vi "test_Move to 0 with Return Speed.vi"(8 "error in (no error)":errorcluster, 11 "TestCase in":refnum<class "EM1000 Turn Table.lvclass">) -> (0 "error out":errorcluster, 3 "TestCase out":refnum<class "EM1000 Turn Table.lvclass">)   [LabVIEW 2020, in "EM1000 Turn Table.lvclass"]
uses:
  EM1000 Turn Table.lvclass
  EM1000 Turn Table.lvclass/EM1000 Turn Table.ctl
  <vilib>/addons/_JKI Toolkits/VI Tester/TestCase.llb/TestCase.lvclass
  AUDIX EM1000.lvclass
  C:/Program Files (x86)/National Instruments/LabVIEW 2020/vi.lib/addons/_JKI Toolkits/VI Tester/TestCase.llb/TestCase.lvclass
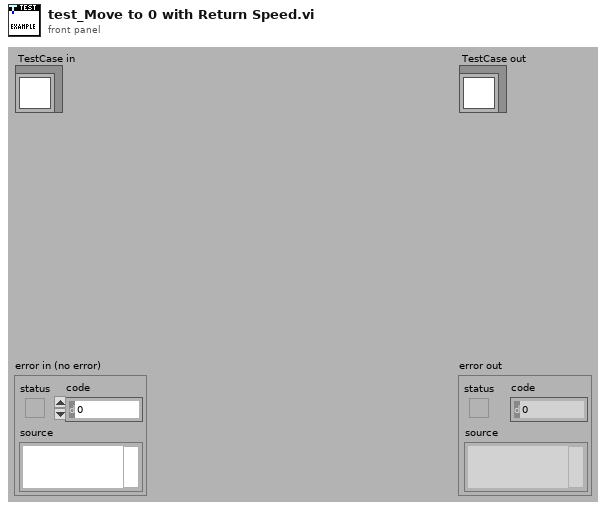
[diagram p1: front panel]
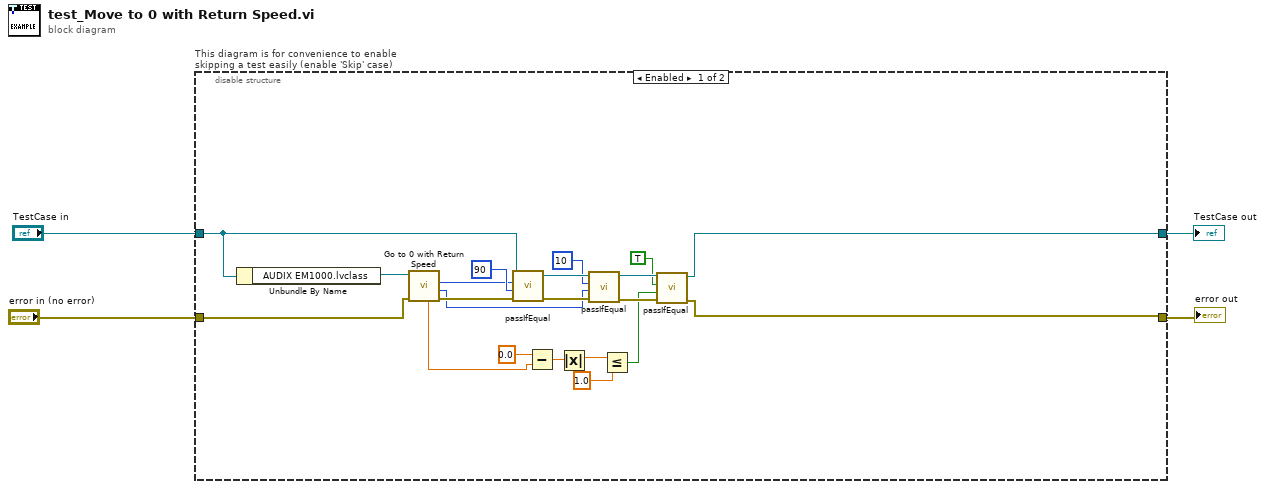
[diagram p0: block diagram]
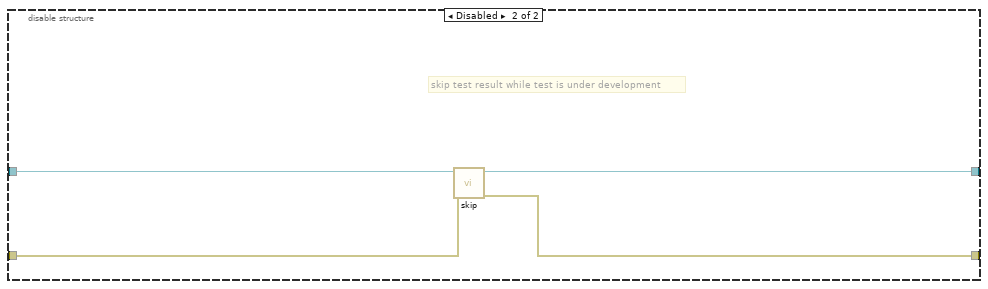
[diagram p2: hidden frame]
diagram:
  n1 = disable-structure "This diagram is for convenience to enable skipping a test easily (enable 'Skip' case)" shown="Enabled" {
    disable-tunnel: "TestCase in" -> [w19 w29]
    disable-tunnel: [w18 w27] -> w1
    disable-tunnel: [w17 w28] -> w3
    disable-tunnel: "error in (no error)" -> [w15 w26]
    frame Enabled {
      n2 = Unbundle By Name(w19) -> ("AUDIX EM1000.lvclass"=w16:refnum<class "AUDIX EM1000.lvclass">)
      n3 = call "Go to 0 with Return Speed.vi"("error in (no error)"=w15, "AUDIX EM1000 in"=w16) -> ("error out"=w14:errorcluster, "Final Speed"=w13:i32, "Return Speed"=w12:i32, "TT Angle"=w7:dbl)  [unwired: 5 in, 1 out]
      n4 = call-dynamic "passIfEqual.vi"("error in (no error)"=w14, "y"=90, "x"=w12, "TestCase in"=w19) -> ("error out"=w21:errorcluster, "TestCase out"=w24:refnum<class "EM1000 Turn Table.lvclass">)  [unwired: 6 in]
      n5 = Subtract(x=0.0, y=w7) -> (x-y=w9:dbl)
      n6 = Absolute Value(x=w9) -> (abs(x)=w10:dbl)
      n7 = call-dynamic "passIfEqual.vi"("error in (no error)"=w21, "y"=w13, "x"=10, "TestCase in"=w24) -> ("error out"=w20:errorcluster, "TestCase out"=w22:refnum<class "EM1000 Turn Table.lvclass">)  [unwired: 6 in]
      n8 = Less Or Equal?(x=w10, y=1.0) -> (x <= y?=w6:bool)
      n9 = call-dynamic "passIfEqual.vi"("error in (no error)"=w20, "y"=w6, "x"=TRUE, "TestCase in"=w22) -> ("error out"=w17:errorcluster, "TestCase out"=w18:refnum<class "EM1000 Turn Table.lvclass">)  [unwired: 6 in]
    }
    frame Disabled {
      # "skip test result while test is under development"
      n10 = call <vilib>:"skip.vi"("error in (no error)"=w26, "TestCase in"=w29) -> ("error out"=w28:errorcluster, "TestCase out"=w27:refnum<class "EM1000 Turn Table.lvclass">)  [unwired: 8 in]
    }
  }
  "error out" <- w3
  "TestCase out" <- w1
